vi "GET-Load.vi"(8 "error in (no error)":errorcluster, 10 "ApiKey":string, 11 "BaseUrl":string) -> (0 "error out":errorcluster, 3 "OpenTool Json":string)   [LabVIEW 2017]
uses:
  <vilib>/httpClient/LabVIEWHTTPClient.lvlib
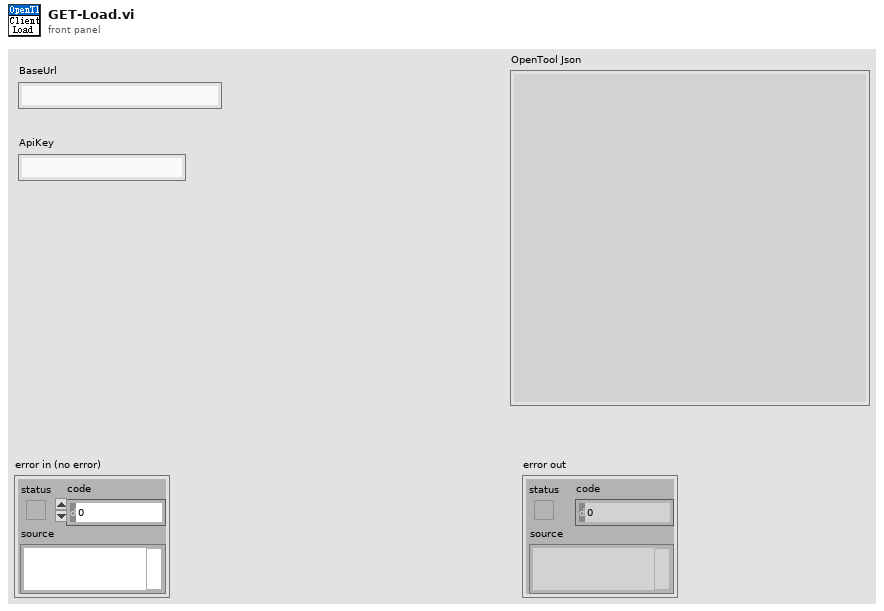
[diagram p1: front panel]
types:
  T1 = typedef "LabVIEWHTTPClient.lvlib/ClientHandle.ctl" = refnum<k1>
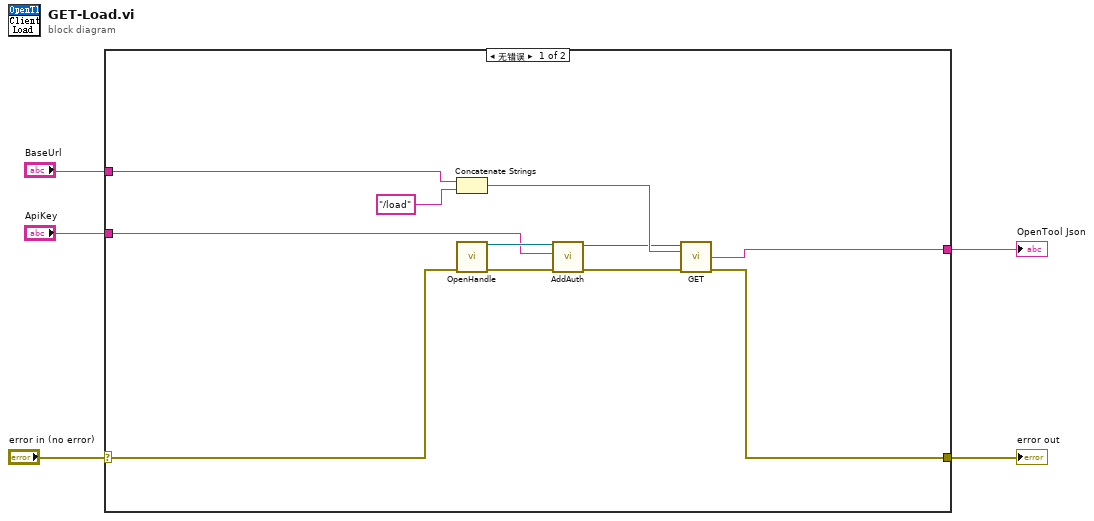
[diagram p0: block diagram]
diagram:
  n1 = case shown="无错误" "error in (no error)" {
    selector: "error in (no error)" -> [w11 w17]
    tunnel: [w13 w17] -> w4
    tunnel: "BaseUrl" -> [w14 _]
    tunnel: [w12 _] -> w2
    tunnel: "ApiKey" -> [w8 _]
    frame No Error {
      n2 = Concatenate Strings(w14, "/load" ("url")) -> (w15:string)
      n3 = call <vilib>:"OpenHandle.vi"("error in (no error)"=w11) -> ("client handle out"=w9:T1, "error out"=w10:errorcluster)  [unwired: 13 in]
      n4 = call "AddAuth.vi"("error in (no error)"=w10, "ApiKey"=w8, "client handle in"=w9) -> ("error out"=w7:errorcluster, "client handle out"=w6:T1)  [unwired: 7 in]
      n5 = call <vilib>:"GET.vi"("client handle"=w6, "url"=w15, "error in (no error)"=w7) -> ("body"=w12:string, "error out"=w13:errorcluster)  [unwired: 9 in, 2 out]
    }
    frame Error {
    }
  }
  "error out" <- w4
  "OpenTool Json" <- w2
